vi "Dedicated Empty Path.vi"(11 "error in":errorcluster) -> (4 "path text":string, 15 "error out":errorcluster)   [LabVIEW 2024]
doc: "Fixture containing the dedicated Empty Path constant."
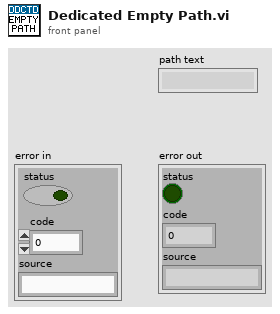
[diagram p1: front panel]
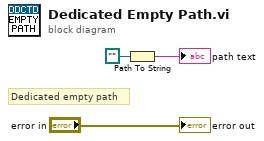
[diagram p0: block diagram]
diagram:
  # "Dedicated empty path"
  n1 = Path To String(path=path "") -> (string=→"path text":string)
  "error out" <- "error in"
